vi "PAQ_BIN_Read_Index.vi"(8 "error in (no error)":errorcluster, 10 "TableName":string, 11 "Path":path) -> (0 "error out":errorcluster, 3 "TimeStamps":T1(array[cluster]))   [LabVIEW 2020, in "Sgraph_lib_V1.lvlib" / "DBAL-BIN.lvclass"]
doc: "Read the index file of a specific layer on disk"
uses:
  DBAL-BIN.lvclass
  DBAL-BIN.lvclass/DBAL-BIN.ctl
panel:
  out "Cluster":T2
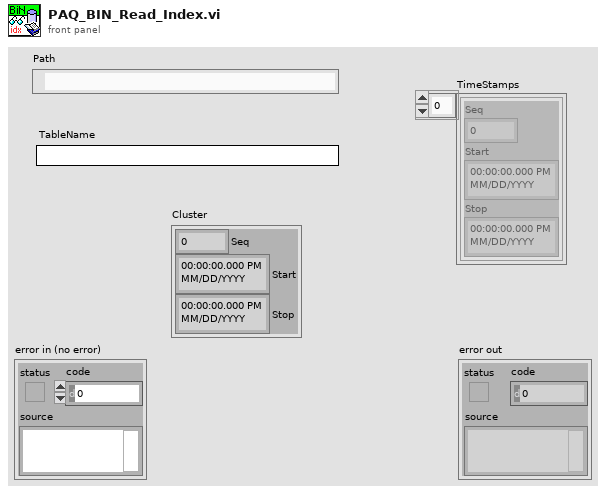
[diagram p1: front panel]
types:
  T1 = cluster{"Seq":i32, "Start":timestamp, "Stop":timestamp}[]
  T2 = cluster{"Seq":dbl, "Start":timestamp, "Stop":timestamp}
  T3 = cluster{"Seq":i32, "Start":timestamp, "Stop":timestamp}
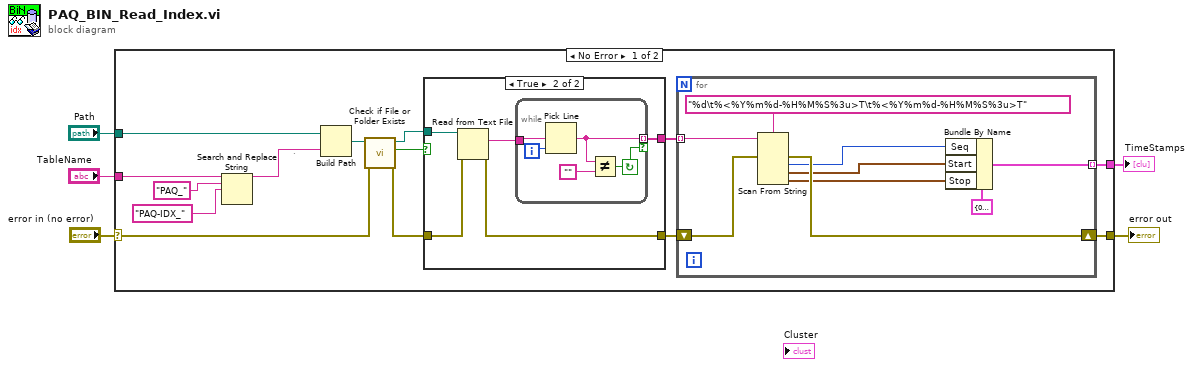
[diagram p0: block diagram]
diagram:
  n1 = case shown="No Error" "error in (no error)" {
    selector: "error in (no error)" -> [w14 w40]
    tunnel: [w6 w40] -> w4
    tunnel: "TableName" -> [w17 _]
    tunnel: "Path" -> [w16 _]
    tunnel: [w9 _] -> w1
    frame No Error {
      # "`"
      n2 = Search and Replace String(input string=w17, search string="PAQ_", replace string="PAQ-IDX_" ("search string")) -> (result string=w8:string)  [unwired: 5 in, 3 out]
      n3 = Build Path(base path=w16, name or relative path=w8) -> (appended path=w15:path)
      n4 = call <vilib>:"Check if File or Folder Exists.vi"("error in (no error)"=w14, "path"=w15) -> ("error out"=w11:errorcluster, "file or folder exists?"=w13:bool, "dup path"=w12:path)  [unwired: 7 in]
      n5 = case shown="True" w13 {
        tunnel: w12 -> [_ w34]
        tunnel: w11 -> [w29 w33]
        tunnel: [w29 w32] -> w7
        tunnel: [_ w30] -> w10
        frame False {
        }
        frame True {
          n6 = Read from Text File(file (use dialog)=w34, error in=w33) -> (text=w31:string, error out=w32:errorcluster)  [unwired: 2 in, 2 out]
          n7 = while {
            tunnel: w31 -> [w39]
            tunnel: [w37] -> w30 mode=indexing if=w35
            i -> [w38]
            stop <- w35 continue-if-true
            n8 = Pick Line(multi-line string=w39, line index=w38) -> (output string=w37:string)  [unwired: 1 in]
            n9 = Not Equal?(x=w37, y="") -> (x != y?=w35:bool)
          }
        }
      }
      n10 = for {
        tunnel: w10 -> [w28] mode=indexing
        tunnel: [w24] -> w9 mode=indexing
        shift-right: [w25] -> w6
        shift-left: w7 -> [w26]
        n11 = Scan From String(format string="%d\t%<%Y%m%d-%H%M%S%3u>T\t%<%Y%m%d-%H%M%S%3u>T", input string=w28, error in=w26) -> (error out=w25:errorcluster, output 1=w20:i32, output 2=w21:timestamp, output 3=w22:timestamp)  [unwired: 4 in, 2 out]
        n12 = Bundle By Name(cluster=T3 {"Seq"=0, "Start"=timestamp(0 s since 1904-01-01), "Stop"=timestamp(0 s since 1904-01-01)} ("Cluster"), "Seq"=w20, "Start"=w21, "Stop"=w22) -> (w24:T3)
      }
    }
    frame Error {
    }
  }
  "error out" <- w4
  "TimeStamps" <- w1
